vi "PI_speed_model_test.vi"() -> ()   [LabVIEW 2020]
uses:
  <vilib>/Platform/TimedLoop/XDataNode/timing_clust.ctl
  <vilib>/Platform/TimedLoop/XDataNode/nitl_modes.ctl
  <vilib>/Platform/TimedLoop/XDataNode/wakeup.ctl
  <vilib>/xnet/xnet.llb/XNET Read (Signal Single-point).vi
  <vilib>/xnet/xnet.llb/XNET Write (Signal Single-point).vi
  <vilib>/Utility/file.llb/Write Delimited Spreadsheet (DBL).vi
  <vilib>/Platform/TimedLoop/XDataNode/XDataNode.xnode
  <vilib>/Platform/TimedLoop/XDataNode/XDNodeRunTimeDep.lvlib
panel:
  out "error out 5":errorcluster caption="write"
  out "Ctrol_time_ms":dbl
  out "Time (s)":dbl
  out "Heartbeat":dbl
  out "Fault":dbl
  out "error out 3":errorcluster
  out "error out 2":errorcluster
  out "error out":errorcluster
  out "Number Output":i16 min=0
  out "Number Input":i16
  out "CarSim Output Data(Vx)":dbl[](array[numeric]) format="%.2f"
  in  "error in (no error)":errorcluster
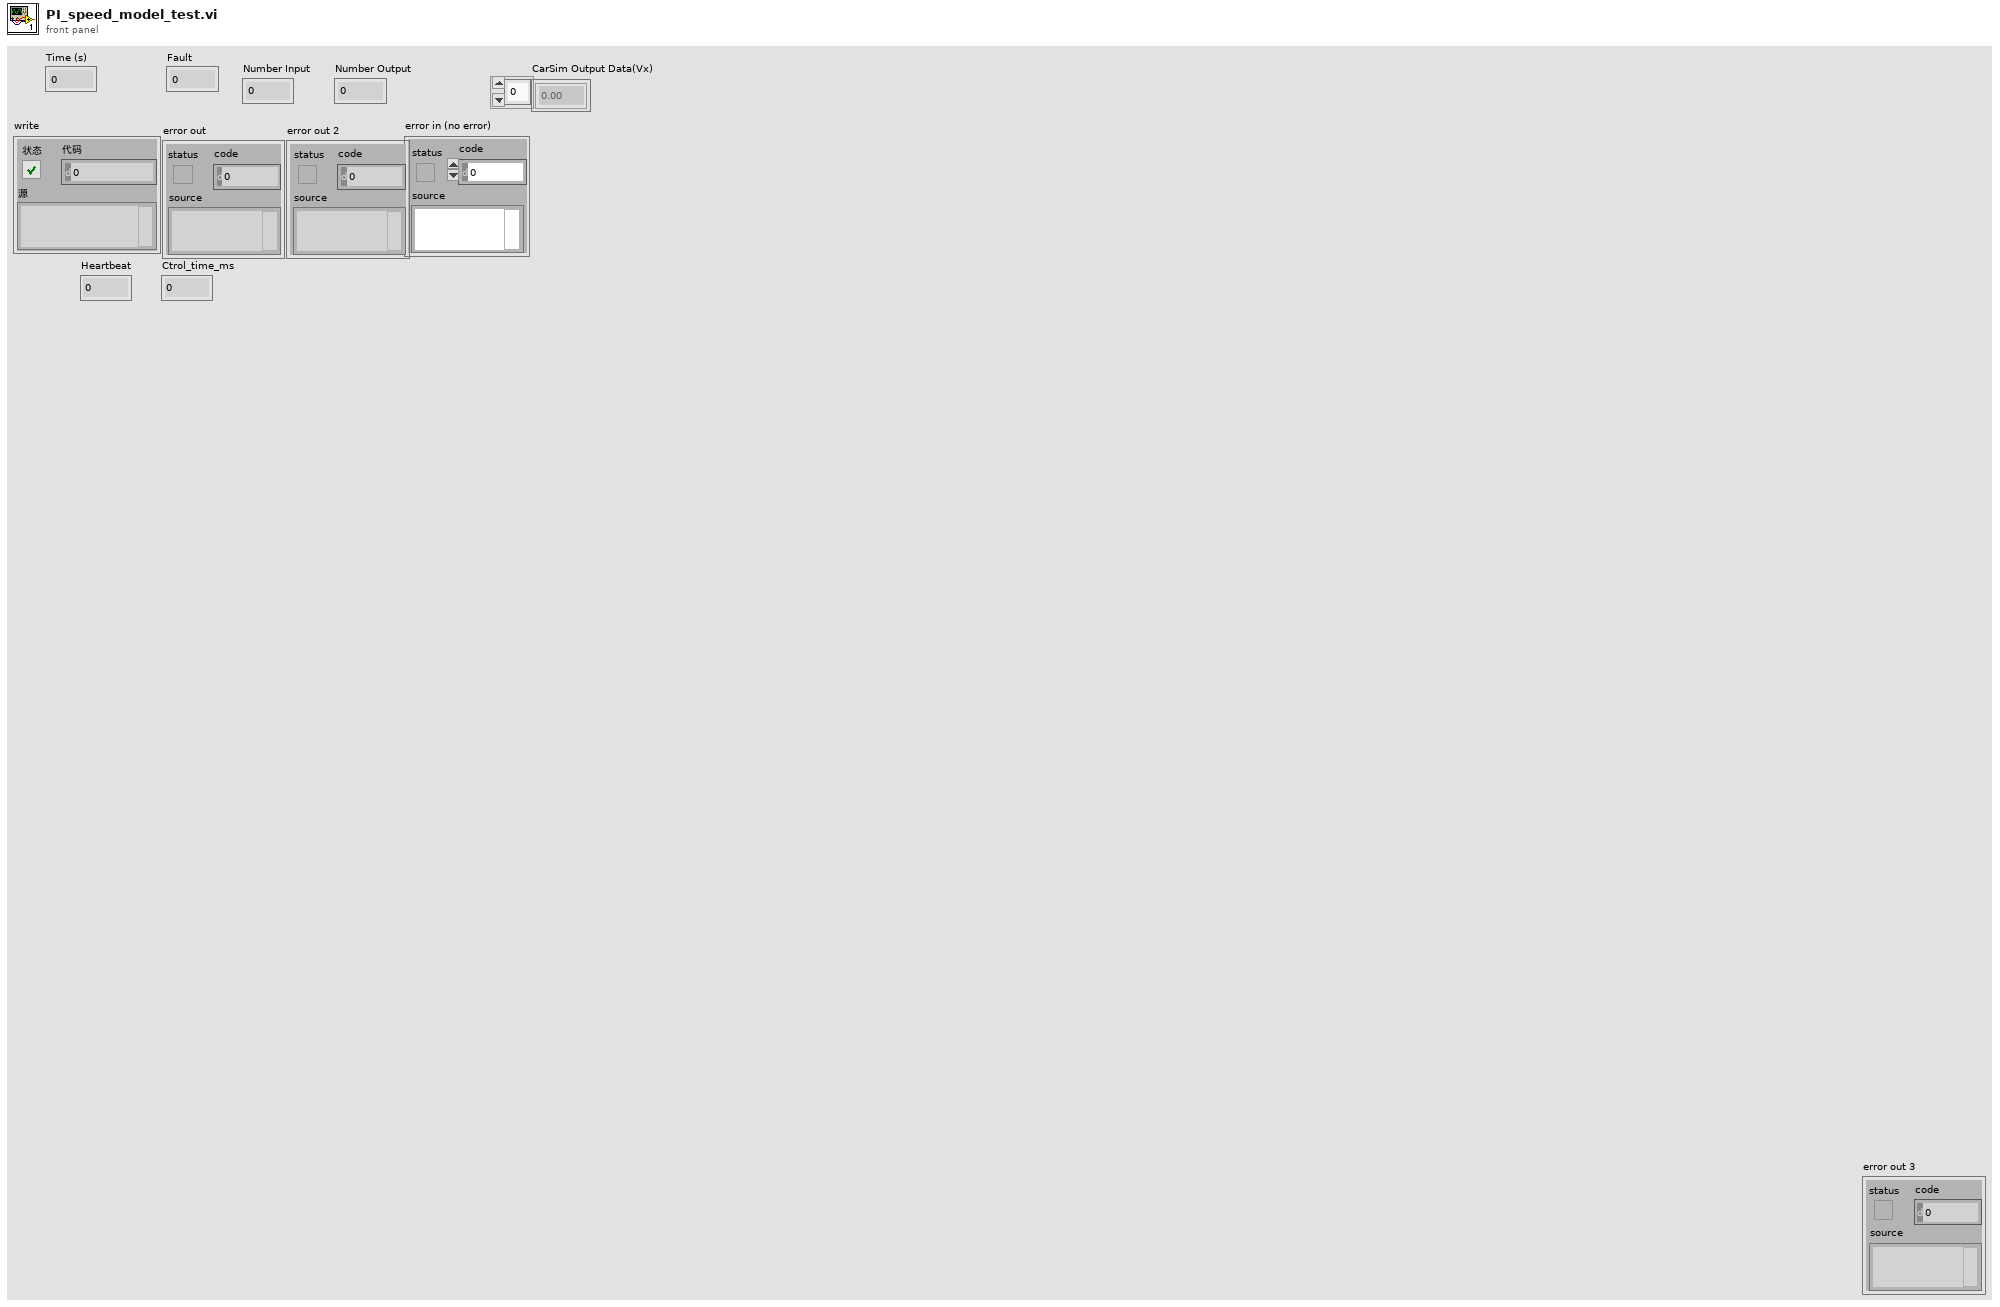
[diagram p1: front panel]
types:
  T1 = typedef "XDNodeRunTimeDep.lvlib/timing_clust.ctl" = cluster{"Expected End [f-1]":u64, "Actual End [f-1]":u64, "Finished Late? [f-1]":bool, "Expected End [i-1]":u64, "Actual End [i-1]":u64, "Finished Late? [i-1]":bool, "Expected Start [i]":u64, "Actual Start [i]":u64, "Expected Start [f]":u64, "Actual Start [f]":u64, "Source Name":string, "Structure Name":string, "Period":i64, "Deadline":i64, "Offset":i64, "Start":i64, "Priority":i32, "Timeout":i32, "Mode":T2, "Wakeup Reason":T3, "Error":errorcluster, "Source Type":string, "Secondary Source Type":string, "Global End Time":u64, "Global Start Time":u64, "Frame Duration":u64, "Iteration Duration":u64, "Assigned CPU":i32, "I/O Scan Engine Mode":u32}
  T2 = typedef "XDNodeRunTimeDep.lvlib/nitl_modes.ctl" = enum32{"No Change", "Process missed periods, maintain original phase", "Discard missed periods, maintain original phase", "Process missed periods, ignore original phase", "Discard missed periods, ignore original phase"}
  T3 = typedef "XDNodeRunTimeDep.lvlib/wakeup.ctl" = enum32{"Normal", "Aborted", "Asynchronous wakeup", "Timing source error", "Timed loop error", "Timeout"}
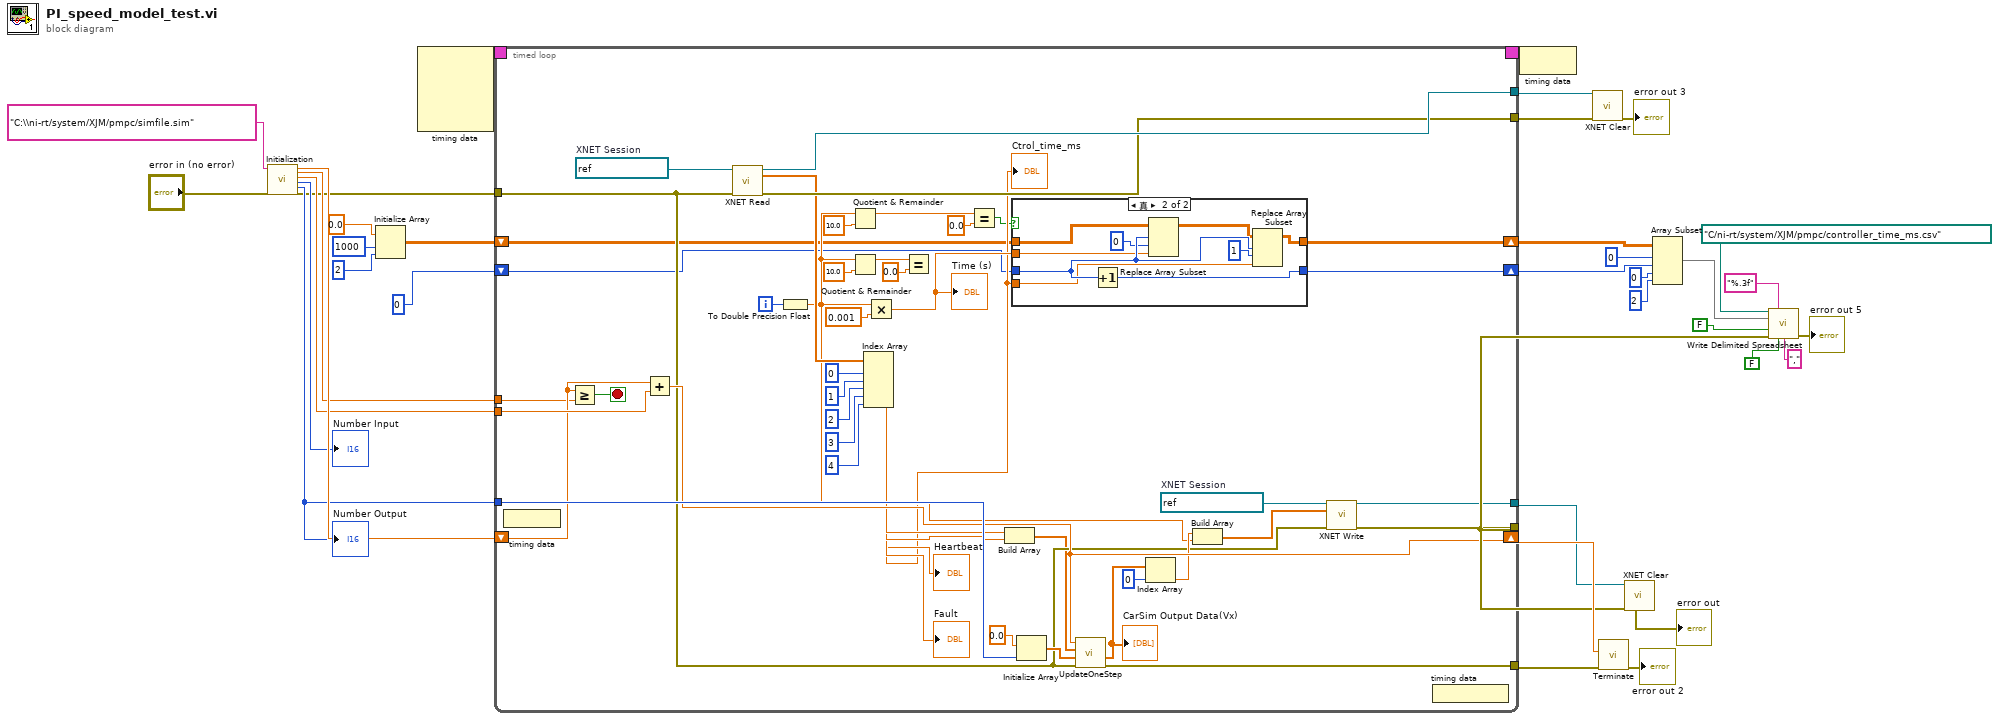
[diagram p0: block diagram]
diagram:
  n1 = call "Initialization.vi"("Simfile"="C:\\ni-rt/system/XJM/pmpc/simfile.sim", "error in (no error)"="error in (no error)") -> ("Start Time"=w34:dbl, "Stop Time"=w29:dbl, "Time Step"=w28:dbl, "Number Input"=→"Number Input":i16, "Number Output"=w33:i16, "error out"=w26:errorcluster)  [unwired: 12 in]
  "Number Output" <- w33
  n2 = Initialize Array(0.0 ("元素"), 1000 ("维数大小"), 2 ("维数大小")) -> (w17:dbl[][])
  n3 = node-c288() -> (w31:T1)  [unwired: 4 in]
  n4 = timed-loop {
    shift-right: [w78] -> w32
    shift-left: w34 -> [w79]
    tunnel: w28 -> [w83]
    tunnel: w33 -> [w81]
    timing: w31 -> [_]
    timing-out: [_] -> w30
    tunnel: [w75] -> w25
    tunnel: w26 -> [w65]
    tunnel: w29 -> [w76]
    tunnel: [w68] -> w24
    tunnel: [w67] -> w5
    tunnel: [w66] -> w20
    tunnel: [w64] -> w19
    shift-right: [w37] -> w13
    shift-left: w17 -> [w38]
    shift-right: [w39] -> w10
    shift-left: 0 -> [w40]
    i -> [w53]
    stop <- w77 stop-if-true
    w73 = refnum<k21> "Signal Input"  # XNET Session
    w74 = refnum<k21> "Signal Output"  # XNET Session
    n5 = node-c288() -> ()  [unwired: 1 in]
    n6 = Greater Or Equal?(x=w79, y=w76) -> (x >= y?=w77:bool)
    n7 = Add(x=w79, y=w83) -> (x+y=w78:dbl)
    n8 = call-poly <vilib>:"XNET Read.vi"("session in"=w73, "error in (no error)"=w65) -> ("session out"=w66:refnum<k21>, "data"=w63:dbl[], "error out"=w64:errorcluster)  [unwired: 11 in]
    n9 = To Double Precision Float(number=w53) -> (double precision float=w47:dbl)
    n10 = Quotient & Remainder(x=w47, y=10.0) -> (x-y*floor(x/y)=w44:dbl)  [unwired: 1 out]
    n11 = Quotient & Remainder(x=w47, y=10.0) -> (x-y*floor(x/y)=w50:dbl)  [unwired: 1 out]
    n12 = Index Array(array=w63, index #1=0, index #2=1, index #3=2, index #4=3, index #5=4) -> (element #1=w58:dbl, element #2=w57:dbl, element #3=→"Heartbeat":dbl, element #4=→"Fault":dbl, element #5=w42:dbl)
    "Ctrol_time_ms" <- w42
    n13 = Multiply(x=w47, y=0.001) -> (x*y=w43:dbl)
    "Time (s)" <- w43
    n14 = Equal?(x=w50, y=0.0) -> ()  [unwired: 1 out]
    n15 = Equal?(x=w44, y=0.0) -> (x = y?=w41:bool)
    n16 = Build Array(w58, w57) -> (w54:dbl[])
    n17 = case shown="真" w41 {
      tunnel: w43 -> [_ w92]
      tunnel: w42 -> [_ w91]
      tunnel: w40 -> [w84 w93]
      tunnel: [w84 w94] -> w39
      tunnel: w38 -> [w85 w88]
      tunnel: [w85 w87] -> w37
      frame False {
      }
      frame True {
        n18 = Increment(x=w93) -> (x+1=w94:i32)
        n19 = Replace Array Subset(array=w88, new element=w92, index (row)=w93, index (col)=0 ("索引 (列)")) -> (w86:dbl[][])
        n20 = Replace Array Subset(array=w86, new element=w91, index (row)=w93, index (col)=1 ("索引 (列)")) -> (w87:dbl[][])
      }
    }
    n21 = Initialize Array(0.0 ("元素"), w81) -> (w80:dbl[])
    n22 = call "UpdateOneStep.vi"("error in (no error)"=w65, "init output"=w80, "input data"=w54, "time"=w78) -> ("error out"=w75:errorcluster, "output data"=w72:dbl[])  [unwired: 5 in, 1 out]
    "CarSim Output Data(Vx)" <- w72
    n23 = Index Array(array=w72, index=0) -> (element=w70:dbl)
    n24 = Build Array(w70, w47) -> (w69:dbl[])
    n25 = call-poly <vilib>:"XNET Write.vi"("session in"=w74, "data"=w69, "error in (no error)"=w65) -> ("session out"=w68:refnum<k21>, "error out"=w67:errorcluster)  [unwired: 11 in]
    n26 = node-c288() -> ()  [unwired: 1 out]
  }
  n27 = node-c288(w30) -> ()
  n28 = call <vilib>:"XNET Clear.vi"("session in"=w20, "error in (no error)"=w19) -> ("error out"=→"error out 3":errorcluster)  [unwired: 13 in]
  n29 = call "Terminate.vi"("error in (no error)"=w25, "time"=w32) -> ("error out"=→"error out 2":errorcluster)  [unwired: 9 in]
  n30 = call <vilib>:"XNET Clear.vi"("session in"=w24, "error in (no error)"=w5) -> ("error out"=→"error out":errorcluster)  [unwired: 13 in]
  n31 = Array Subset(array=w13, index (row)=0 ("索引"), length (row)=w10, index (col)=0 ("索引"), length (col)=2 ("长度")) -> (w12:dbl[][])
  n32 = call-poly <vilib>:"Write Delimited Spreadsheet.vi"("file path (dialog if empty)"=path "C:/ni-rt/system/XJM/pmpc/controller_time_ms.csv", "format (%.3f)"="%.3f", "2D data"=w12, "append to file? (new file:F)"=FALSE, "error in (no error)"=w5, "transpose? (no:F)"=FALSE, "delimiter (\\t)"="," ("delimiter (\\t)")) -> ("error out"=→"error out 5":errorcluster)  [unwired: 7 in, 1 out]
